vi "Get Children ALL.vi"(8 "error in":errorcluster, 9 "pure children？":bool, 10 "Parent Tag":string, 11 "Tree Reference":refnum<vi>) -> (0 "error out":errorcluster, 2 "Children Tags":string[](array[string]), 3 "Tree Reference":refnum<vi>)   [LabVIEW 2023, in "DSLV_Tree.lvlib"]
uses:
  DSLV_Tree.lvlib
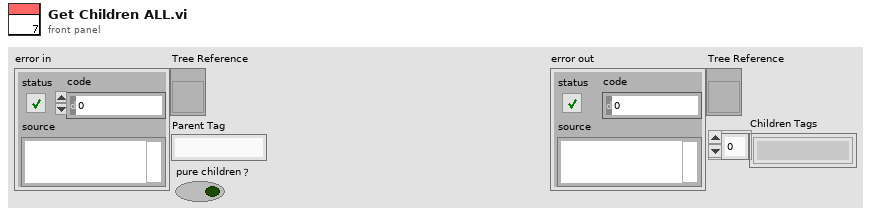
[diagram p1: front panel]
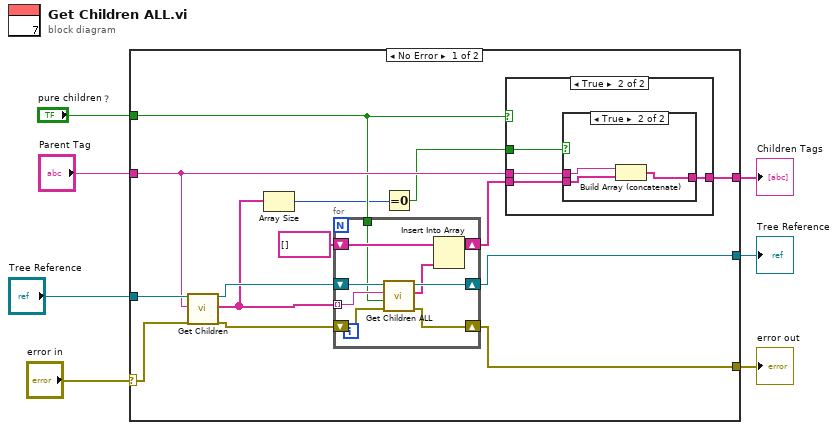
[diagram p0: block diagram]
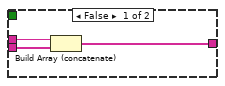
[diagram p2: hidden frame]
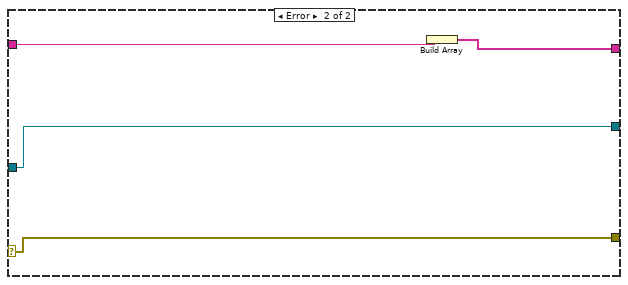
[diagram p4: hidden frame]
diagram:
  n1 = case shown="No Error" "error in" {
    selector: "error in" -> [w12 w42]
    tunnel: [w21 w42] -> w7
    tunnel: [w20 w43] -> w6
    tunnel: "Tree Reference" -> [w19 w43]
    tunnel: "Parent Tag" -> [w18 w45]
    tunnel: [w16 w44] -> w3
    tunnel: "pure children？" -> [w11 _]
    frame No Error {
      n2 = call "Get Children.vi"("Tree Reference In"=w19, "Parent Tag"=w18, "error in (no error)"=w12) -> ("Tree Reference Out"=w15:refnum<vi>, "Children Tags"=w10:string[], "error out"=w13:errorcluster)  [unwired: 14 in]
      n3 = Array Size(array=w10) -> (size(s)=w9:i32)
      n4 = for {
        shift-right: [w41] -> w20
        shift-left: w15 -> [w40]
        shift-right: [w39] -> w21
        shift-left: w13 -> [w38]
        tunnel: w10 -> [w37] mode=indexing
        shift-right: [w35] -> w17
        shift-left: string[] [] -> [w34]
        tunnel: w11 -> [w33]
        n5 = call "Get Children ALL.vi"("error in"=w38, "pure children？"=w33, "Parent Tag"=w37, "Tree Reference"=w40) -> ("error out"=w39:errorcluster, "Children Tags"=w36:string[], "Tree Reference"=w41:refnum<vi>)  [unwired: 5 in]
        n6 = Insert Into Array(array=w34, new element=w36) -> (w35:string[])  [unwired: 1 in]
      }
      n7 = Equal To 0?(x=w9) -> (x = 0?=w8:bool)
      n8 = case shown="True" w11 {
        tunnel: w18 -> [w24 w26]
        tunnel: w17 -> [w23 w27]
        tunnel: [w22 w25] -> w16
        tunnel: w8 -> [_ w28]
        frame False {
          n9 = Build Array (concatenate)(w24, w23) -> (w22:string[])
        }
        frame True {
          n10 = case shown="True" w28 {
            tunnel: w27 -> [w29 w32]
            tunnel: w26 -> [_ w31]
            tunnel: [w29 w30] -> w25
            frame False {
            }
            frame True {
              n11 = Build Array (concatenate)(w31, w32) -> (w30:string[])
            }
          }
        }
      }
    }
    frame Error {
      n12 = Build Array(w45) -> (w44:string[])
    }
  }
  "error out" <- w7
  "Tree Reference" <- w6
  "Children Tags" <- w3
